vi "For_Loop_Array_Statistics.vi"() -> ()   [LabVIEW 2026]
panel:
  out "Average":i32
  out "Minimum":dbl format="%.2f"
  out "Maximum":dbl format="%.2f"
  in  "Input Numeric Array":dbl[](array[numeric])
  out "Sum":i32
  # "Array Statistics Calculator"
  # "Calculate Sum, Maximum, Minimum and Average using For Loop"
  # "Results"
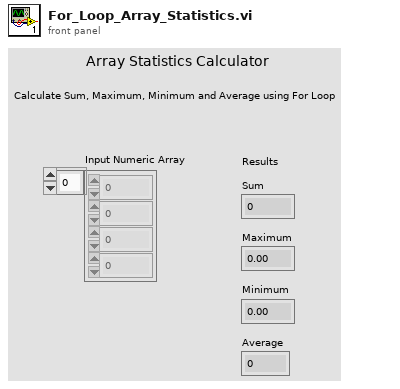
[diagram p1: front panel]
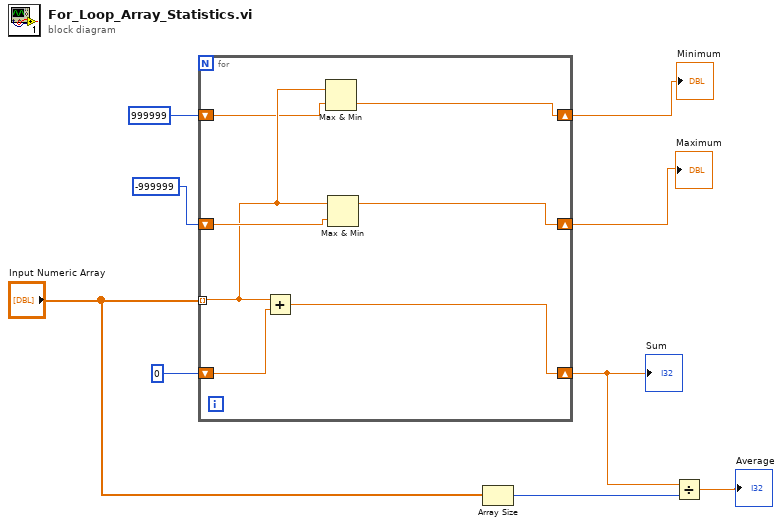
[diagram p0: block diagram]
diagram:
  n1 = for {
    shift-right: [w15] -> w3
    shift-left: 0 -> [w16]
    tunnel: "Input Numeric Array" -> [w12] mode=indexing
    shift-right: [w13] -> w7
    shift-left: -999999 -> [w14]
    shift-right: [w10] -> w5
    shift-left: 999999 -> [w11]
    n2 = Add(x=w12, y=w16) -> (x+y=w15:dbl)
    n3 = Max & Min(x=w12, y=w11) -> (min(x,y)=w10:dbl)  [unwired: 1 out]
    n4 = Max & Min(x=w12, y=w14) -> (max(x,y)=w13:dbl)  [unwired: 1 out]
  }
  "Sum" <- w3
  "Maximum" <- w7
  "Minimum" <- w5
  n5 = Array Size(array="Input Numeric Array") -> (size(s)=w2:i32)
  n6 = Divide(x=w3, y=w2) -> (x/y=→"Average":dbl)
